vi "Rocket_DAQ_Main.vi"() -> ()   [LabVIEW 2026]
uses:
  <vilib>/Utility/file.llb/Write Delimited Spreadsheet (DBL).vi
  <vilib>/Analysis/NI_AALPro.lvlib
panel:
  out "Dominant freq Hz":dbl
  out "Abort reason":string
  out "State name":string
  out "FFT amplitude spectrum (1 bin = 10 Hz)":dbl[](graph)
  in  "stop":bool
  out "HF waveform of FFT channel":dbl[](graph)
  out "HF RMS [25]":dbl[](array[numeric])
  out "DIO [60]":dbl[](array[numeric])
  out "Slow ch raw V [50]":dbl[](array[numeric])
  out "Slow ch scaled [50]":dbl[](array[numeric])
  out "Abort time s":dbl
  out "Abort code":dbl
  out "Fuel valve V":dbl
  out "Ox valve V":dbl
  out "Thrust N":dbl
  out "Chamber pressure bar":dbl(graph)
  out "Mixture ratio":dbl
  out "Total flow kg/s":dbl
  out "Time s":dbl
  out "State":dbl
  in  "FFT channel":dbl
  in  "Hold time s":dbl
  in  "Abort limit bar":dbl
  in  "Target MR":dbl
  in  "Target flow kg/s":dbl
  in  "Fault inject":dbl
  in  "E-Stop 0/1":dbl
  in  "Command":dbl
  # "SIMULATION ONLY - no hardware is driven. Demonstration values.\nCommand: 1 start test (pre-check)   2 start sequence   3 stop   4 reset   5 manual abort\nState: 0 IDLE  1 PRE-CHECK  2 READY  3 START  4 RAMP  5 HOLD  6 SHUTDOWN  7 COMPLETE  8 ABORT\nFault inject: 0 none  1 chamber overpressure  2 PT-07 disconnected  3 PT-07 stuck  4 tank overpressure  7 HF instability tone\nAbort code: 1 overpressure (any pressure channel)  2 sensor out of range  3 sensor stale  4 E-stop  5 no ignition  6 manual\nPressure limits: chamber channels use Abort limit bar; tank and line channels use 50 bar"
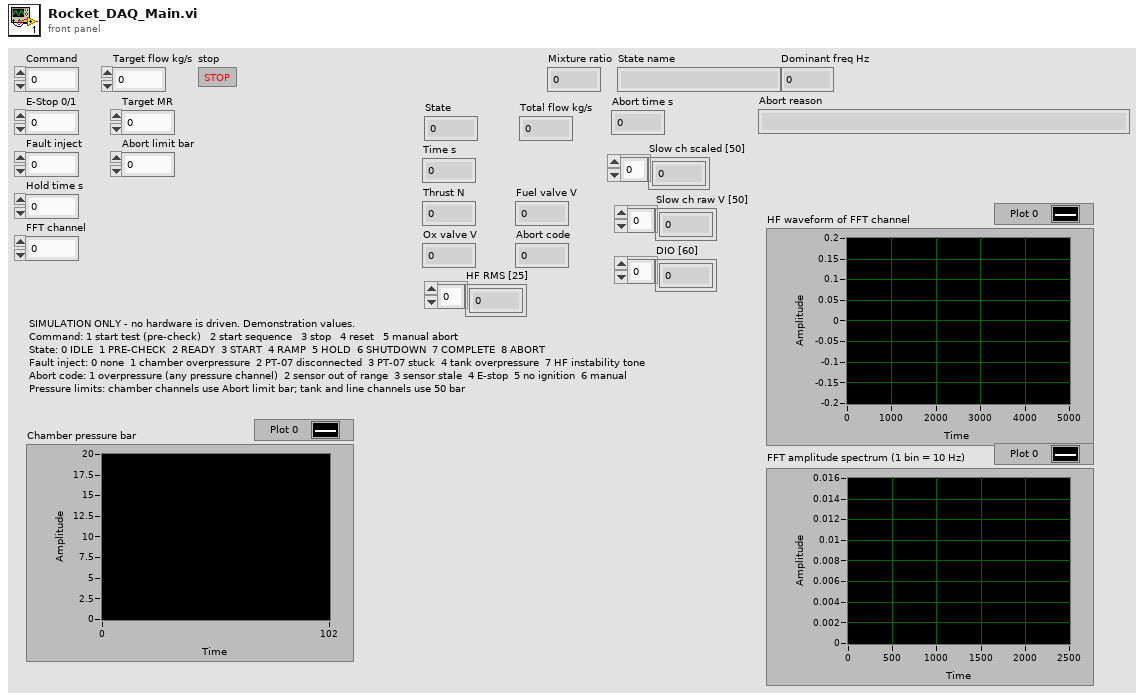
[diagram p1: front panel]
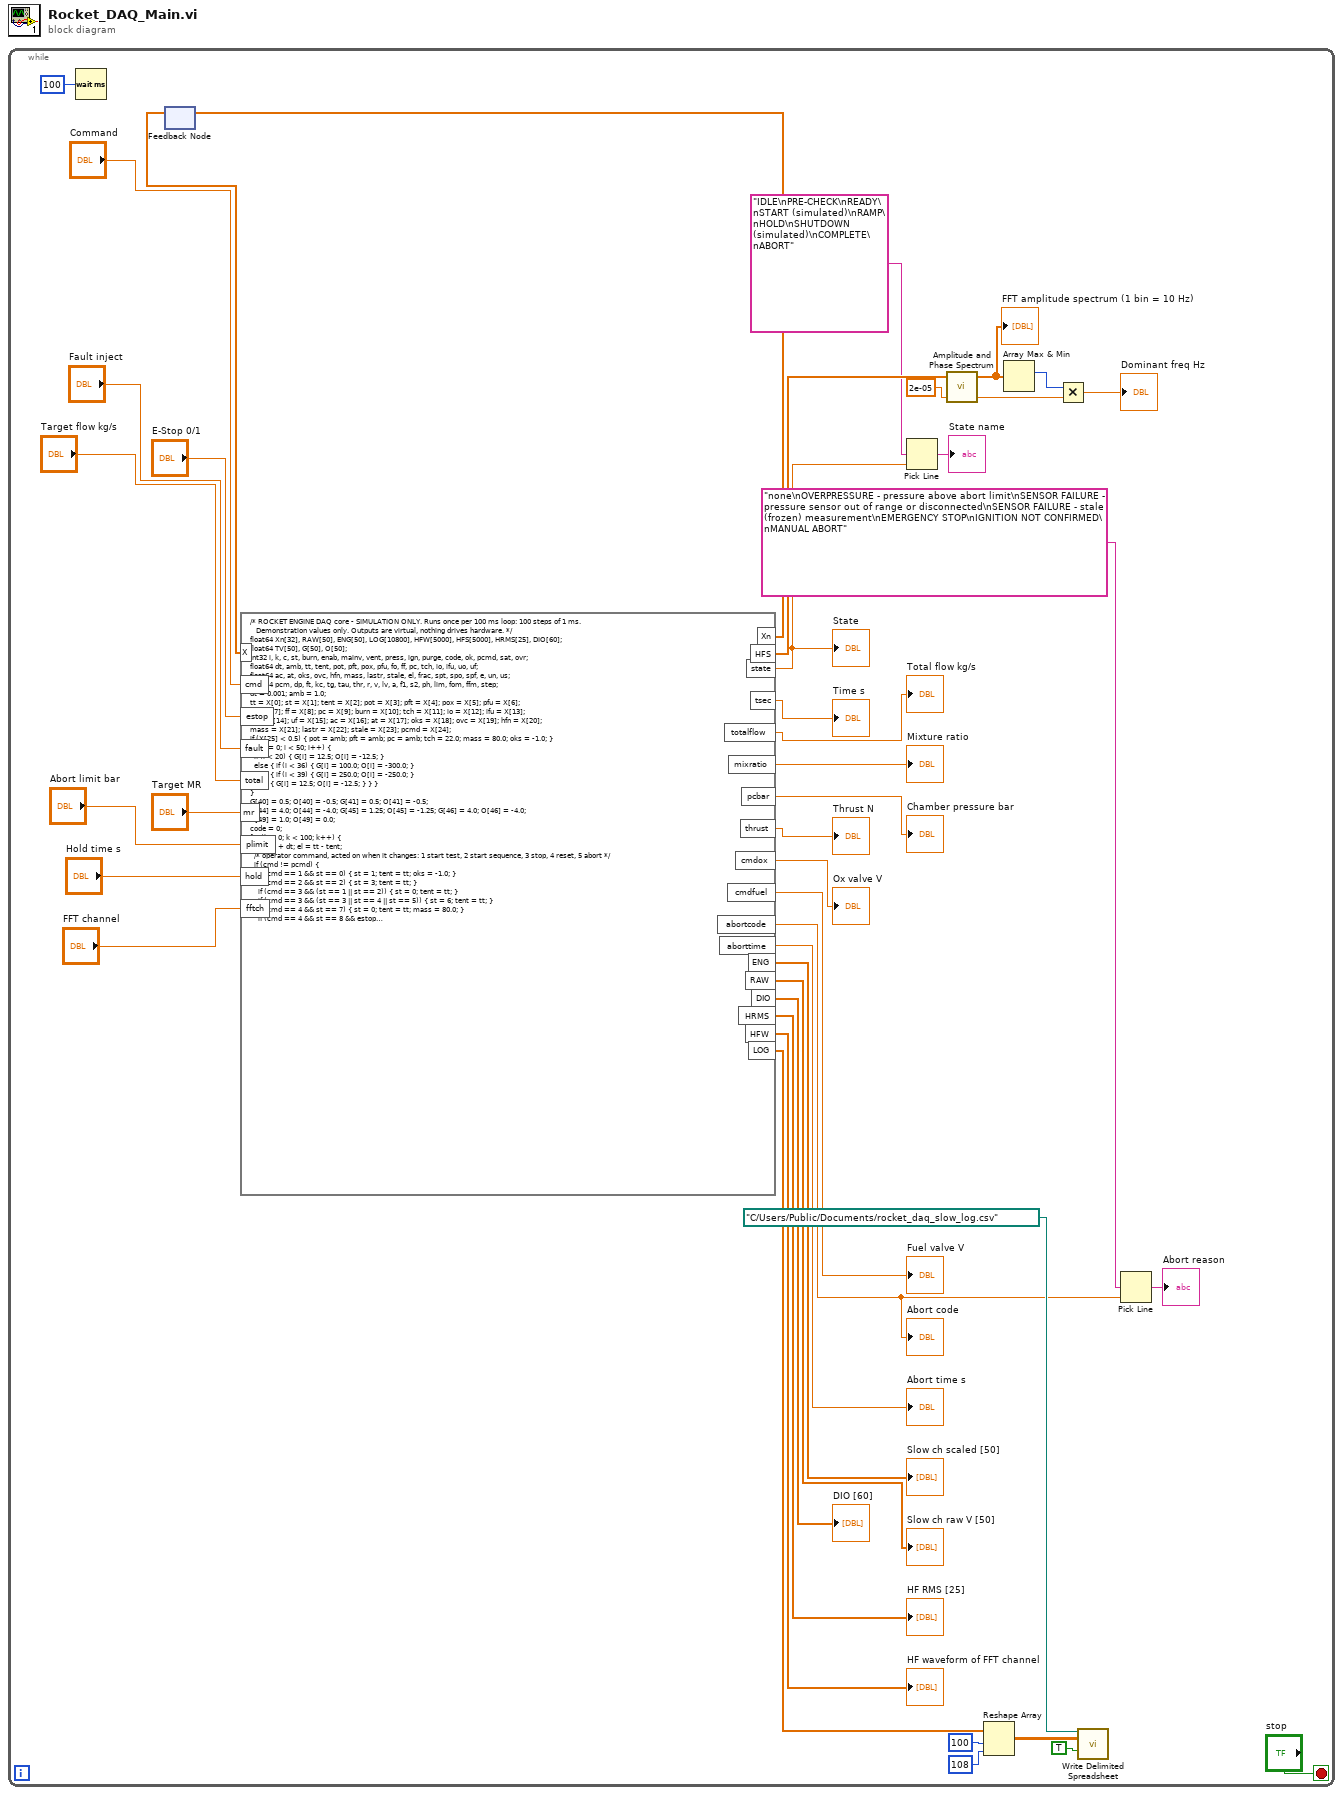
[diagram p0: block diagram]
diagram:
  n1 = while {
    stop <- "stop" stop-if-true
    n2 = Wait (ms)(milliseconds to wait=u32 100) -> ()  [unwired: 1 out]
    n3 = feedback #1() -> (w21:dbl[])  [unwired: 1 in]
    n4 = formula code="/* ROCKET ENGINE DAQ core - SIMULATION ONLY. Runs once per 100 ms loop: 100 steps of 1 ms.\n   Demonstration values only. Outputs are virtual, nothing drives hardware. */\nfloat64 Xn[32], RAW[50], ENG[50], LOG[10800], HFW[5000], HFS[5000], HRMS[25], DIO[60];\nfloat64 TV[50], G[50], O[50];\nint32 i, k, c, st, burn, enab, mainv, vent, press, ign, purge, code, ok, pcmd, sat, ovr;\nfloat64 dt, amb, tt, tent, pot, pft, pox, pfu, fo, ff, pc, tch, io, ifu, uo, uf;\nfloat64 ac, at, oks, ovc, hfn, mass, lastr, stale, el, frac, spt, spo, spf, e, un, us;\nfloat64 pcm, dp, ft, kc, tg, tau, thr, r, v, lv, a, f1, s2, ph, lim, fom, ffm, step;\ndt = 0.001; amb = 1.0;\ntt = X[0]; st = X[1]; tent = X[2]; pot = X[3]; pft = X[4]; pox = X[5]; pfu = X[6];\nfo = X[7]; ff = X[8]; pc = X[9]; burn = X[10]; tch = X[11]; io = X[12]; ifu = X[13];\nuo = X[14]; uf = X[15]; ac = X[16]; at = X[17]; oks = X[18]; ovc = X[19]; hfn = X[20];\nmass = X[21]; lastr = X[22]; stale = X[23]; pcmd = X[24];\nif (X[25] < 0.5) { pot = amb; pft = amb; pc = amb; tch = 22.0; mass = 80.0; oks = -1.0; }\nfor (i = 0; i < 50; i++) {\n  if (i < 20) { G[i] = 12.5; O[i] = -12.5; }\n  else { if (i < 36) { G[i] = 100.0; O[i] = -300.0; }\n  else { if (i < 39) { G[i] = 250.0; O[i] = -250.0; }\n  else { G[i] = 12.5; O[i] = -12.5; } } }\n}\nG[40] = 0.5; O[40] = -0.5; G[41] = 0.5; O[41] = -0.5;\nG[44] = 4.0; O[44] = -4.0; G[45] = 1.25; O[45] = -1.25; G[46] = 4.0; O[46] = -4.0;\nG[49] = 1.0; O[49] = 0.0;\ncode = 0;\nfor (k = 0; k < 100; k++) {\n  tt = tt + dt; el = tt - tent;\n  /* operator command, acted on when it changes: 1 start test, 2 start sequence, 3 stop, 4 reset, 5 abort */\n  if (cmd != pcmd) {\n    if (cmd == 1 && st == 0) { st = 1; tent = tt; oks = -1.0; }\n    if (cmd == 2 && st == 2) { st = 3; tent = tt; }\n    if (cmd == 3 && (st == 1 || st == 2)) { st = 0; tent = tt; }\n    if (cmd == 3 && (st == 3 || st == 4 || st == 5)) { st = 6; tent = tt; }\n    if (cmd == 4 && st == 7) { st = 0; tent = tt; mass = 80.0; }\n    if (cmd == 4 && st == 8 && estop < 0.5 && fault < 0.5) { st = 0; tent = tt; ac = 0.0; at = 0.0; mass = 80.0; }\n    if (cmd == 5 && st != 8) { code = 6; }\n    pcmd = cmd;\n  }\n  el = tt - tent;\n  /* sequencer timing */\n  if (st == 3 && el >= 2.0) { if (pc < 3.0) { code = 5; } else { st = 4; tent = tt; el = 0.0; } }\n  if (st == 4 && el >= 3.0) { st = 5; tent = tt; el = 0.0; }\n  if (st == 5 && el >= hold) { st = 6; tent = tt; el = 0.0; }\n  if (st == 6 && el >= 3.0) { st = 7; tent = tt; el = 0.0; }\n  el = tt - tent;\n  /* virtual outputs for the current state */\n  press = (st >= 1 && st <= 5);\n  vent = (st == 0 || st == 7 || st == 8 || (st == 6 && el >= 2.0));\n  ign = (st == 3 && el >= 0.4);\n  mainv = ((st == 3 && el >= 0.8) || st == 4 || st == 5 || (st == 6 && el < 1.0));\n  purge = ((st == 3 && el < 0.3) || st == 6 || st == 8);\n  enab = ((st == 3 && el >= 0.8) || st == 4 || st == 5);\n  frac = 1.0;\n  if (st == 3) { frac = 0.3; }\n  if (st == 4) { frac = 0.3 + 0.7 * el / 3.0; }\n  /* simulated plant */\n  if (vent) { pot = pot + (amb - pot) * dt / 1.2; pft = pft + (amb - pft) * dt / 1.2; }\n  else { if (press) { pot = pot + (40.0 - pot) * dt / 0.6; pft = pft + (40.0 - pft) * dt / 0.6; } }\n  pox = pox + (uo / 10.0 - pox) * dt / 0.12;\n  pfu = pfu + (uf / 10.0 - pfu) * dt / 0.12;\n  dp = pot - 0.8 * fo - pc; if (dp < 0.0) { dp = 0.0; }\n  ft = 3.2 * pox * mainv * sqrt(dp / 20.0);\n  fo = fo + (ft - fo) * dt / 0.05;\n  dp = pft - 0.8 * ff - pc; if (dp < 0.0) { dp = 0.0; }\n  ft = 1.6 * pfu * mainv * sqrt(dp / 20.0);\n  ff = ff + (ft - ff) * dt / 0.05;\n  mass = mass - (fo + ff) * dt;\n  if (ign && fo > 0.1 && ff > 0.05) { burn = 1; }\n  if (burn && (fo < 0.05 || ff < 0.03)) { burn = 0; }\n  kc = 0.6; if (burn) { kc = 7.6; }\n  pc = pc + (amb + kc * (fo + ff) - pc) * dt / 0.03;\n  pcm = pc; if (fault == 1) { pcm = pc + 15.0; }\n  tg = 22.0; if (burn) { tg = 22.0 + 26.0 * (pc - amb); }\n  tau = 9.0; if (tg > tch) { tau = 3.0; }\n  tch = tch + (tg - tch) * dt / tau;\n  thr = 158.0 * (pcm - amb); if (thr < 0.0) { thr = 0.0; } if (!burn) { thr = thr * 0.05; }\n  /* true values of the 50 slow channels */\n  TV[0] = pot; if (fault == 4) { TV[0] = pot + 15.0; } TV[1] = pft; TV[2] = pot - 1.4 * fo; TV[3] = pft - 1.4 * ff;\n  TV[4] = pcm * 1.05; TV[5] = pcm * 1.05; TV[6] = pcm; TV[7] = pcm;\n  TV[8] = 1.0 + 14.0 * purge; TV[9] = 8.0; TV[10] = pot * 1.02 + 0.3; TV[11] = pft * 1.02 + 0.3;\n  TV[12] = 0.99 * (pot - 1.4 * fo); TV[13] = 0.99 * (pft - 1.4 * ff); TV[14] = 0.95 * pcm;\n  TV[15] = 0.55 * pcm + 0.45; TV[16] = 4.8; TV[17] = 3.6; TV[18] = amb; TV[19] = amb;\n  for (i = 20; i < 36; i++) { TV[i] = 22.0 + (tch - 22.0) * (36 - i) / 16.0; }\n  TV[36] = thr / 3.0; TV[37] = thr / 3.0; TV[38] = thr / 3.0; TV[39] = mass;\n  TV[40] = fo; TV[41] = ff; TV[42] = 100.0 * pox; TV[43] = 100.0 * pfu;\n  TV[44] = 24.0; TV[45] = 1.5; TV[46] = 1.0 + 24.0 * ign; TV[47] = 45.0; TV[48] = 2.0; TV[49] = 5.0;\n  /* sensors: true value -> raw volts (+ noise, faults) -> SCALING: eng = raw * gain + offset */\n  for (i = 0; i < 50; i++) {\n    r = (TV[i] - O[i]) / G[i] + 0.004 * (rand() + rand() + rand() - 1.5);\n    if (i == 6 && fault == 2) { r = 0.01 + 0.002 * rand(); }\n    if (i == 6 && fault == 3) { r = lastr; }\n    RAW[i] = r;\n    ENG[i] = r * G[i] + O[i];\n  }\n  if (RAW[6] == lastr) { stale = stale + 1.0; } else { stale = 0.0; }\n  lastr = RAW[6];\n  /* safety monitor */\n  ok = 1;\n  for (i = 0; i < 20; i++) {\n    if (RAW[i] < 0.5 || RAW[i] > 9.8) { ok = 0; if (st >= 2 && st <= 6 && code == 0) { code = 2; } }\n  }\n  if (stale >= 500.0) { ok = 0; if (st >= 2 && st <= 6 && code == 0) { code = 3; } }\n  /* overpressure: EVERY pressure channel is checked against its limit.\n     chamber channels (PT-07, PT-08, PT-15, PT-16) use the operator limit,\n     tank, line and injector channels use 50 bar */\n  ovr = 0;\n  for (i = 0; i < 20; i++) {\n    lim = 50.0;\n    if (i == 6 || i == 7 || i == 14 || i == 15) { lim = plimit; }\n    if (ENG[i] > lim) { ovr = 1; }\n  }\n  if (ovr) { ovc = ovc + 1.0; } else { ovc = 0.0; }\n  if (ovc >= 3.0 && st >= 2 && st <= 6 && code == 0) { code = 1; }\n  if (estop > 0.5 && code == 0) { code = 4; }\n  if (code != 0 && st != 8) { st = 8; tent = tt; ac = code; at = tt; uo = 0.0; uf = 0.0; io = 0.0; ifu = 0.0; enab = 0; }\n  /* pre-check */\n  if (st == 1) {\n    if (ok && ENG[0] > 35.0 && ENG[0] < 45.0 && ENG[1] > 35.0 && ENG[1] < 45.0 && ENG[6] < 2.5 && estop < 0.5) {\n      if (oks < 0.0) { oks = tt; } else { if (tt - oks >= 1.0) { st = 2; tent = tt; } }\n    } else { oks = -1.0; if (el > 10.0) { st = 0; tent = tt; } }\n  }\n  /* flow controller: total flow and mixture ratio -> one PI loop per valve */\n  fom = ENG[40]; ffm = ENG[41];\n  step = 20.0 * dt;\n  if (enab) {\n    spt = total * frac; spo = spt * mr / (1.0 + mr); spf = spt / (1.0 + mr);\n    e = spo - fom; un = 2.5 * e + io + 22.0 * e * dt;\n    us = un; if (us > 10.0) { us = 10.0; } if (us < 0.0) { us = 0.0; }\n    sat = (us != un);\n    if (us > uo + step) { us = uo + step; sat = 1; } if (us < uo - step) { us = uo - step; sat = 1; }\n    if (!sat || (un > us && e < 0.0) || (un < us && e > 0.0)) { io = io + 22.0 * e * dt; }\n    if (io > 10.0) { io = 10.0; } if (io < 0.0) { io = 0.0; }\n    uo = us;\n    e = spf - ffm; un = 5.0 * e + ifu + 44.0 * e * dt;\n    us = un; if (us > 10.0) { us = 10.0; } if (us < 0.0) { us = 0.0; }\n    sat = (us != un);\n    if (us > uf + step) { us = uf + step; sat = 1; } if (us < uf - step) { us = uf - step; sat = 1; }\n    if (!sat || (un > us && e < 0.0) || (un < us && e > 0.0)) { ifu = ifu + 44.0 * e * dt; }\n    if (ifu > 10.0) { ifu = 10.0; } if (ifu < 0.0) { ifu = 0.0; }\n    uf = us;\n  } else {\n    spt = 0.0;\n    uo = uo - step; if (uo < 0.0) { uo = 0.0; }\n    uf = uf - step; if (uf < 0.0) { uf = 0.0; }\n    io = uo; ifu = uf;\n  }\n  /* log row: time, state, abort code, set-point, flows, valve commands, 50 raw, 50 scaled */\n  c = k * 108;\n  LOG[c] = tt; LOG[c + 1] = st; LOG[c + 2] = ac; LOG[c + 3] = spt; LOG[c + 4] = fom; LOG[c + 5] = ffm;\n  LOG[c + 6] = uo; LOG[c + 7] = uf;\n  for (i = 0; i < 50; i++) { LOG[c + 8 + i] = RAW[i]; LOG[c + 58 + i] = ENG[i]; }\n}\n/* 25 high-frequency channels, 5000 samples each (50 kS/s for 100 ms).\n   HFS = selected channel with a Hann window (amplitude corrected) for the FFT */\nlv = 0.0; if (burn) { lv = (pc - amb) / 19.0; }\nfor (c = 0; c < 25; c++) {\n  if (c < 10) { f1 = 1200.0 + 35.0 * c; } else { if (c < 20) { f1 = 800.0 + 20.0 * (c - 10); } else { f1 = 1000.0 + 500.0 * (24 - c); } }\n  a = 0.02 + 0.98 * lv; if (c == 24) { a = 1.0; }\n  s2 = 0.0;\n  for (i = 0; i < 5000; i++) {\n    ph = 2.0 * pi * (hfn + i) / 50000.0;\n    v = a * sin(f1 * ph) + 0.4 * a * sin(2.0 * f1 * ph) + 0.1 * (rand() + rand() + rand() - 1.5);\n    if (fault == 7 && c < 20) { v = v + 3.0 * sin(1850.0 * ph); }\n    s2 = s2 + v * v;\n    if (c == fftch) { HFW[i] = v; HFS[i] = v * (1.0 - cos(2.0 * pi * i / 5000.0)); }\n  }\n  HRMS[c] = sqrt(s2 / 5000.0);\n}\nhfn = hfn + 5000.0;\n/* digital inputs 0..29 and virtual digital outputs 30..59 */\nfor (i = 0; i < 60; i++) { DIO[i] = 0.0; }\nDIO[0] = (estop < 0.5); DIO[1] = 1.0; DIO[2] = 1.0; DIO[3] = 1.0; DIO[4] = 1.0; DIO[5] = 1.0;\nDIO[6] = mainv; DIO[7] = !mainv; DIO[8] = mainv; DIO[9] = !mainv; DIO[10] = vent; DIO[11] = !vent;\nDIO[12] = vent; DIO[13] = !vent; DIO[14] = purge; DIO[15] = !purge; DIO[16] = press; DIO[17] = !press;\nDIO[20] = (pc > 3.0); DIO[21] = burn;\nDIO[30] = mainv; DIO[31] = mainv; DIO[32] = vent; DIO[33] = vent; DIO[34] = purge; DIO[35] = press;\nDIO[36] = press; DIO[37] = ign; DIO[39] = (st >= 2 && st != 7); DIO[43] = (st == 8);\n/* outputs */\nstate = st; tsec = tt; totalflow = fom + ffm; mixratio = 0.0; if (ffm > 0.02) { mixratio = fom / ffm; }\npcbar = ENG[6]; cmdox = uo; cmdfuel = uf; abortcode = ac; aborttime = at; thrust = ENG[36] + ENG[37] + ENG[38];\nXn[0] = tt; Xn[1] = st; Xn[2] = tent; Xn[3] = pot; Xn[4] = pft; Xn[5] = pox; Xn[6] = pfu;\nXn[7] = fo; Xn[8] = ff; Xn[9] = pc; Xn[10] = burn; Xn[11] = tch; Xn[12] = io; Xn[13] = ifu;\nXn[14] = uo; Xn[15] = uf; Xn[16] = ac; Xn[17] = at; Xn[18] = oks; Xn[19] = ovc; Xn[20] = hfn;\nXn[21] = mass; Xn[22] = lastr; Xn[23] = stale; Xn[24] = pcmd; Xn[25] = 1.0;\nfor (i = 26; i < 32; i++) { Xn[i] = 0.0; }"("cmd"="Command", "estop"="E-Stop 0/1", "fault"="Fault inject", "total"="Target flow kg/s", "mr"="Target MR", "plimit"="Abort limit bar", "hold"="Hold time s", "fftch"="FFT channel", "X"=w21) -> ("Xn"=w22:dbl[], "state"=w9:dbl, "tsec"=→"Time s":dbl, "totalflow"=→"Total flow kg/s":dbl, "mixratio"=→"Mixture ratio":dbl, "pcbar"=→"Chamber pressure bar":dbl, "thrust"=→"Thrust N":dbl, "cmdox"=→"Ox valve V":dbl, "cmdfuel"=→"Fuel valve V":dbl, "abortcode"=w6:dbl, "aborttime"=→"Abort time s":dbl, "ENG"=→"Slow ch scaled [50]":dbl[], "RAW"=→"Slow ch raw V [50]":dbl[], "DIO"=→"DIO [60]":dbl[], "HRMS"=→"HF RMS [25]":dbl[], "HFW"=→"HF waveform of FFT channel":dbl[], "LOG"=w16:dbl[], "HFS"=w12:dbl[])
    "State" <- w9
    "Abort code" <- w6
    n5 = feedback-in #1(w22) -> ()
    n6 = Pick Line(multi-line string="IDLE\nPRE-CHECK\nREADY\nSTART (simulated)\nRAMP\nHOLD\nSHUTDOWN (simulated)\nCOMPLETE\nABORT", line index=w9) -> (output string=→"State name":string)  [unwired: 1 in]
    n7 = call <vilib>:"Amplitude and Phase Spectrum.vi"("dt"=2e-05, "Signal (V)"=w12) -> ("df"=w2:dbl, "Amp Spectrum Mag (Vrms)"=w4:dbl[])  [unwired: 1 in, 1 out]
    "FFT amplitude spectrum (1 bin = 10 Hz)" <- w4
    n8 = Reshape Array(w16, 100 ("dimension size"), 108 ("dimension size")) -> (w15:dbl[][])
    n9 = Array Max & Min(array=w4) -> (max index (indices)=w3:i32)  [unwired: 3 out]
    n10 = Multiply(x=w3, y=w2) -> (x*y=→"Dominant freq Hz":dbl)
    n11 = call-poly <vilib>:"Write Delimited Spreadsheet.vi"("file path (dialog if empty)"=path "C:/Users/Public/Documents/rocket_daq_slow_log.csv", "2D data"=w15, "append to file? (new file:F)"=TRUE) -> ()  [unwired: 11 in, 2 out]
    n12 = Pick Line(multi-line string="none\nOVERPRESSURE - pressure above abort limit\nSENSOR FAILURE - pressure sensor out of range or disconnected\nSENSOR FAILURE - stale (frozen) measurement\nEMERGENCY STOP\nIGNITION NOT CONFIRMED\nMANUAL ABORT", line index=w6) -> (output string=→"Abort reason":string)  [unwired: 1 in]
  }
